vi "optical_snap.vi"() -> ()   [LabVIEW 2025]
uses:
  <vilib>/vision/driver/IMAQdx.llb/IMAQdx Acquisition Mode.ctl
  <vilib>/vision/driver/NI_Vision_Acquisition_Software.lvlib
panel:
  out "Image":T1(plugin-control)
  out "error out":errorcluster
  out "Times between Frames":u32
  in  "Output Folder":path=path "../data/raw/test_2"
  in  "Stop":bool
  in  "Camera Name":refnum<k21> caption="IMAQdx Session"
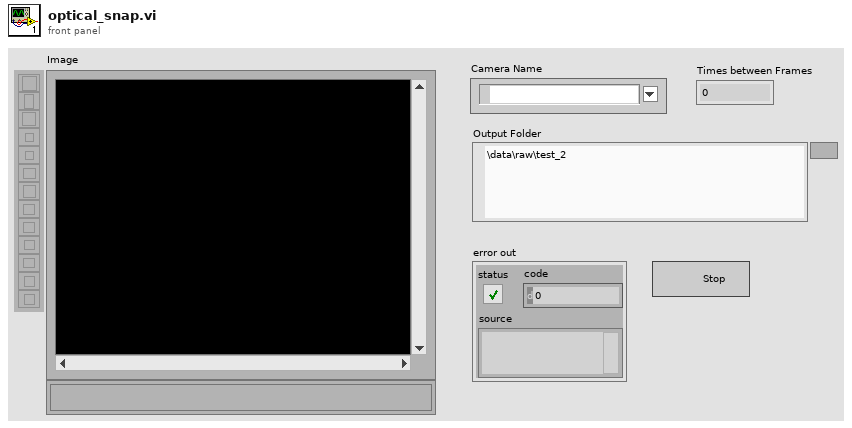
[diagram p1: front panel]
types:
  T1 = typedef "IMAQ Image.ctl" = refnum<image>
  T2 = typedef "Image Type" = u32
  T3 = typedef "NI_Vision_Acquisition_Software.lvlib/IMAQdx Acquisition Mode.ctl" = enum32{"One Shot", "Continuous"}
  T4 = typedef "IMAQdx.ctl" = refnum<k21>
  T5 = enum16{"big-endian, network order", "native, host order", "little-endian"}
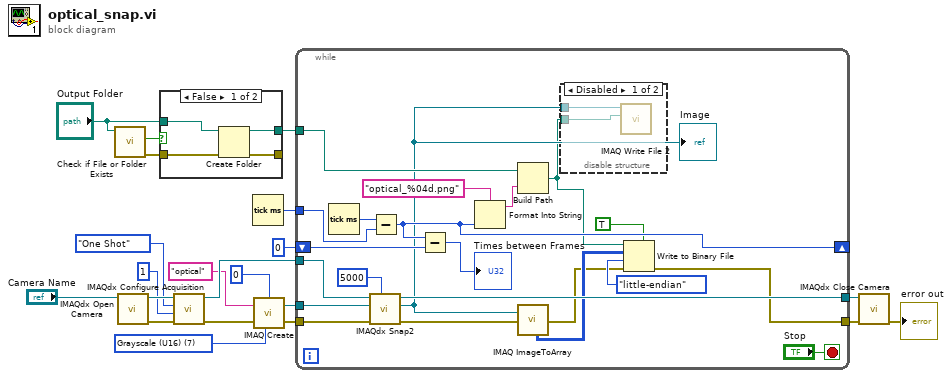
[diagram p0: block diagram]
diagram:
  w2 = T2 7 items=["Grayscale (U8)", "Grayscale (I16)", "Grayscale (SGL)", "Complex (CSG)", "RGB (U32)", "HSL (U32)", "RGB (U64)", "Grayscale (U16)"] ("Image Type")
  n1 = call <vilib>:"Check if File or Folder Exists.vi"("path"="Output Folder") -> ("error out"=w19:errorcluster, "file or folder exists?"=w21:bool)  [unwired: 8 in, 1 out]
  n2 = call <vilib>:"IMAQdx Open Camera.vi"("Session In"="Camera Name") -> ("error out"=w12:errorcluster, "Session Out"=w13:T4)  [unwired: 9 in]
  n3 = case shown="False" w21 {
    tunnel: "Output Folder" -> [w25 w27]
    tunnel: [w24 w27] -> w18
    tunnel: w19 -> [w23 w26]
    tunnel: [w22 w26] -> _
    frame False {
      n4 = Create Folder(path (use dialog)=w25, error in=w23) -> (created path=w24:path, error out=w22:errorcluster)  [unwired: 1 in, 1 out]
    }
    frame True {
    }
  }
  n5 = call <vilib>:"IMAQdx Configure Acquisition.vi"("error in"=w12, "Number of Buffers"=u32 1, "Continuous?"=IMAQdx_Acquisition_Mode."One Shot", "Session In"=w13) -> ("error out"=w5:errorcluster, "Session Out"=w7:T4)  [unwired: 6 in]
  n6 = Tick Count (ms)() -> (millisecond timer value=w17:u32)
  n7 = call "IMAQ Create"("Border Size"=0, "Image Name"="optical", "Image Type"=w2, "error in (no error)"=w5) -> ("New Image"=w6:T1, "error out"=w4:errorcluster)  [unwired: 1 in]
  n8 = while {
    tunnel: w18 -> [w48]
    tunnel: w17 -> [w46]
    shift-right: [w43] -> _
    shift-left: u32 0 -> [w44]
    tunnel: w7 -> [w37]
    tunnel: [w40] -> w15
    tunnel: [w28] -> w14
    tunnel: w4 -> [w39]
    tunnel: w6 -> [w36]
    stop <- "Stop" stop-if-true
    n9 = Tick Count (ms)() -> (millisecond timer value=w47:u32)
    n10 = call <vilib>:"IMAQdx Snap2.vi"("Timeout (ms)"=5000, "error in"=w39, "Image In"=w36, "Session In"=w37) -> ("error out"=w29:errorcluster, "Image Out"=w34:T1, "Session Out"=w40:T4)  [unwired: 5 in]
    "Image" <- w34
    n11 = Subtract(x=w47, y=w46) -> (x-y=w43:u32)
    n12 = Subtract(x=w43, y=w44) -> (x-y=→"Times between Frames":u32)
    n13 = Format Into String(format string="optical_%04d.png", w43) -> (resulting string=w42:string)  [unwired: 2 in, 1 out]
    n14 = Build Path(base path=w48, name or relative path=w42) -> (appended path=w33:path)
    n15 = call "IMAQ ImageToArray"("Image"=w34) -> ("Image Pixels (U16)"=w30:u16[][])  [unwired: 3 in, 4 out]
    n16 = disable-structure shown="Disabled" {
      disable-tunnel: w33 -> [w50 _]
      disable-tunnel: w34 -> [w49 _]
      frame Disabled {
        n17 = call-poly "IMAQ Write File 2"("File Path"=w50, "Image"=w49) -> ()  [unwired: 8 in, 2 out]
      }
      frame Enabled {
      }
    }
    n18 = Write to Binary File(file (use dialog)=w33, data=w30, error in=w29, 5:TRUE ("prepend array or string size? (T)"), 9:T5."little-endian" ("byte order (0:big-endian, network order)")) -> (error out=w28:errorcluster)  [unwired: 1 in, 2 out]
  }
  n19 = call <vilib>:"IMAQdx Close Camera.vi"("error in"=w14, "Session In"=w15) -> ("error out"=→"error out":errorcluster)  [unwired: 9 in]
